vi "DialogCreateClass_FilterAndOrderClassTemplates.vi"(7 "ProviderShortName":string, 8 "error in (no error)":errorcluster, 11 "AllTemplatesForThisProvider/InheritanceType(Base/Sub)":T1[](array[typedef])) -> (0 "error out":errorcluster, 2 "NewOrderIndex":i32[](array[numeric]), 3 "FilteredTemplates":T1[](array[typedef]))   [LabVIEW 2020]
uses:
  <resource>/Framework/Providers/Open_GDS/ClassProviders/Provider_BaseClassInterface/ClassTemplateType.ctl
  <resource>/Framework/Providers/Open_GDS/ClassProviders/Provider_LvNativeClass/ClassWriterNative_class/ClassWriterNative.lvclass
  <resource>/Framework/Providers/Open_GDS/ClassProviders/Provider_BaseClassInterface/ClassWriter_class/ClassWriter.lvclass
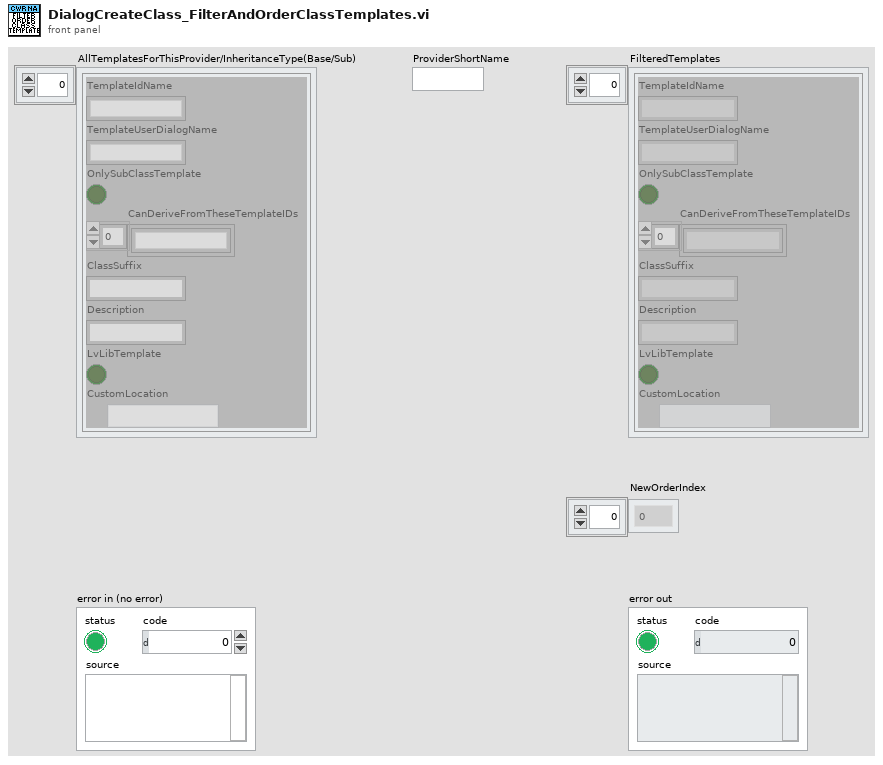
[diagram p1: front panel]
types:
  T1 = typedef "ClassWriter.lvclass/ClassTemplateType.ctl" = cluster{"TemplateIdName":string, "TemplateUserDialogName":string, "OnlySubClassTemplate":bool, "CanDeriveFromTheseTemplateIDs":string[], "ClassSuffix":string, "Description":string, "LvLibTemplate":bool, "CustomLocation":path}
  T2 = cluster{"TemplateNamesSortOrder":string[], "HiddenTemplateNames":string[]}
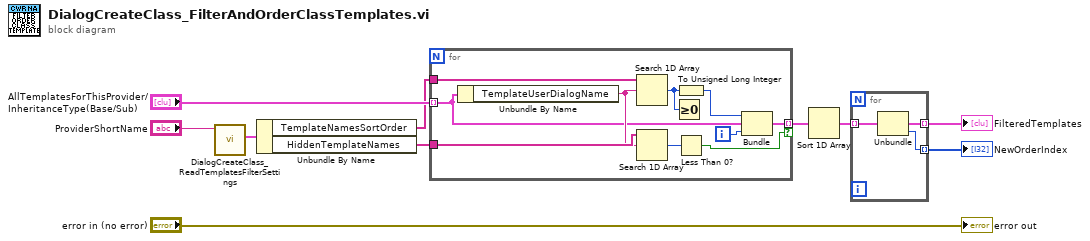
[diagram p0: block diagram]
diagram:
  n1 = call <resource>:"DialogCreateClass_ReadTemplatesFilterSettings.vi"("ProviderShortName"="ProviderShortName") -> ("TemplateFilter"=w8:T2)  [unwired: 9 in, 1 out]
  n2 = Unbundle By Name(w8) -> ("TemplateNamesSortOrder"=w6:string[], "HiddenTemplateNames"=w5:string[])
  n3 = for {
    tunnel: "AllTemplatesForThisProvider/InheritanceType(Base/Sub)" -> [w11] mode=indexing
    tunnel: w6 -> [w20]
    tunnel: [w17] -> w4 mode=indexing if=w13
    tunnel: w5 -> [w16]
    i -> [w12]
    n4 = Unbundle By Name(w11) -> ("TemplateUserDialogName"=w15:string)
    n5 = Search 1D Array(1D array=w20, element=w15) -> (index of element=w19:i32)  [unwired: 1 in]
    n6 = Search 1D Array(1D array=w16, element=w15) -> (index of element=w14:i32)  [unwired: 1 in]
    n7 = Greater Or Equal To 0?(x=w19) -> ()  [unwired: 1 out]
    n8 = To Unsigned Long Integer(number=w19) -> (unsigned 32bit integer=w18:u32)
    n9 = Less Than 0?(x=w14) -> (x < 0?=w13:bool)
    n10 = Bundle(w18, "ClassTemplateType"=w11, w12) -> (w17:cluster{u32, "ClassTemplateType":T1, i32})  [unwired: 1 in]
  }
  n11 = Sort 1D Array(array=w4) -> (sorted array=w3:cluster{u32, "ClassTemplateType":T1, i32}[])
  n12 = for {
    tunnel: w3 -> [w23] mode=indexing
    tunnel: [w22] -> w2 mode=indexing
    tunnel: [w21] -> w1 mode=indexing
    n13 = Unbundle(w23) -> ("ClassTemplateType"=w21:T1, w22:i32)  [unwired: 1 out]
  }
  "FilteredTemplates" <- w1
  "NewOrderIndex" <- w2
  "error out" <- "error in (no error)"
